vi "VIH UI - Property Page VI Refnum Container.vi"(6 "cmd (get)":enum16{"get", "set"}(ring), 11 "VI Refnum":refnum<vi>) -> (0 "active":bool, 3 "VI Refnum out":refnum<vi>)   [LabVIEW 2014]
doc: "::: VI Helpeks :::\nCopyright (c) 2000-2026 Konstantin Shifershteyn. All rights reserved."
panel:
  # "VI Helpeks\nCopyright (c) 2012-2026 Konstantin Shifershteyn"
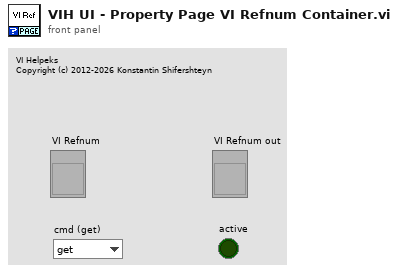
[diagram p1: front panel]
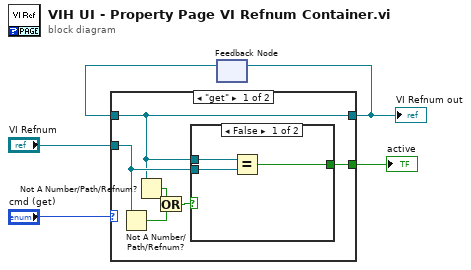
[diagram p0: block diagram]
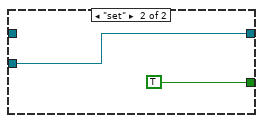
[diagram p3: hidden frame]
diagram:
  n1 = feedback #1() -> (w3:refnum<vi>)  [unwired: 1 in]
  n2 = case shown="\"get\"" "cmd (get)" {
    tunnel: [w7 w16] -> w1
    tunnel: "VI Refnum" -> [w8 w16]
    tunnel: w3 -> [w7 _]
    tunnel: [w6 TRUE] -> w2
    frame "get" {
      n3 = Not A Number/Path/Refnum?(number/path/refnum=w8) -> (NaN/Path/Refnum?=w11:bool)
      n4 = Not A Number/Path/Refnum?(number/path/refnum=w7) -> (NaN/Path/Refnum?=w10:bool)
      n5 = Or(x=w10, y=w11) -> (x .or. y?=w9:bool)
      n6 = case shown="False" w9 {
        tunnel: w8 -> [w14 _]
        tunnel: w7 -> [w13 _]
        tunnel: [w12 _] -> w6
        frame False {
          n7 = Equal?(x=w13, y=w14) -> (x = y?=w12:bool)
        }
        frame True {
        }
      }
    }
    frame "set" {
    }
  }
  "VI Refnum out" <- w1
  "active" <- w2
  n8 = feedback-in #1(w1) -> ()
